vi "test_Antenna Pol Test.vi"(8 "error in (no error)":errorcluster, 11 "TestCase in":refnum<class "CO3000 Test Case.lvclass">) -> (0 "error out":errorcluster, 3 "TestCase out":refnum<class "CO3000 Test Case.lvclass">)   [LabVIEW 2020, in "CO3000 Test Case.lvclass"]
uses:
  CO3000 Test Case.lvclass
  CO3000 Test Case.lvclass/CO3000 Test Case.ctl
  CO3000.lvclass/CO3000.ctl
  CO3000.lvclass
  <vilib>/addons/_JKI Toolkits/VI Tester/TestCase.llb/TestCase.lvclass
  C:/Program Files (x86)/National Instruments/LabVIEW 2020/vi.lib/addons/_JKI Toolkits/VI Tester/TestCase.llb/TestCase.lvclass
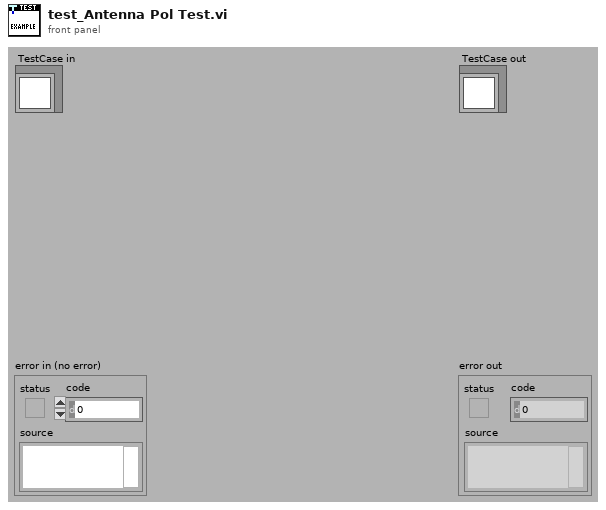
[diagram p1: front panel]
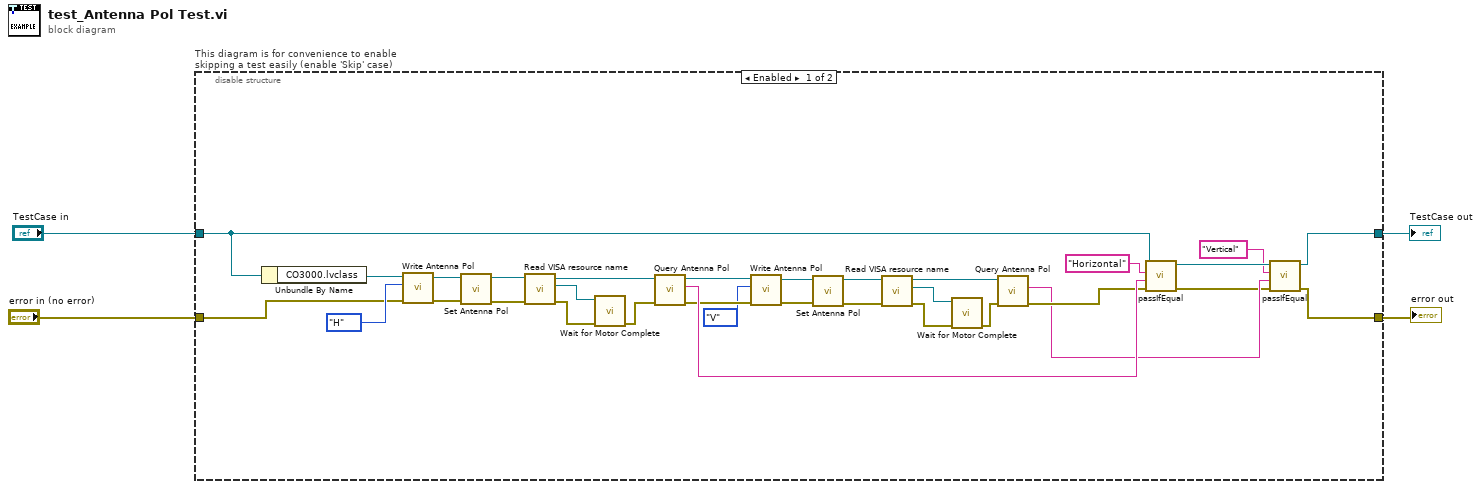
[diagram p0: block diagram]
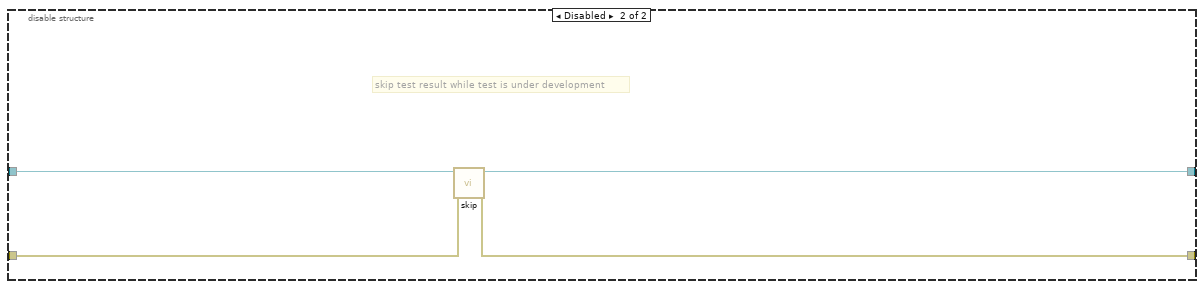
[diagram p2: hidden frame]
diagram:
  n1 = disable-structure "This diagram is for convenience to enable skipping a test easily (enable 'Skip' case)" shown="Enabled" {
    disable-tunnel: "TestCase in" -> [w36 w40]
    disable-tunnel: [w19 w38] -> w1
    disable-tunnel: [w15 w39] -> w3
    disable-tunnel: "error in (no error)" -> [w14 w37]
    frame Enabled {
      n2 = Unbundle By Name(w36) -> ("CO3000.lvclass"=w35:refnum<class "CO3000.lvclass">)
      n3 = call "Write Antenna Pol.vi"("error in (no error)"=w14, "Antenna Pol"=enum16{"H", "V"}."H", "CO3000 in"=w35) -> ("error out"=w32:errorcluster, "CO3000 out"=w33:refnum<class "CO3000.lvclass">)  [unwired: 7 in]
      n4 = call-dynamic "Set Antenna Pol.vi"("error in (no error)"=w32, "CO3000 in"=w33) -> ("error out"=w26:errorcluster, "CO3000 out"=w31:refnum<class "CO3000.lvclass">)  [unwired: 8 in]
      n5 = call "Read VISA resource name.vi"("error in (no error)"=w26, "CO3000 in"=w31) -> ("error out"=w27:errorcluster, "VISA resource name"=w30:refnum<visa-resource-name>, "CO3000 out"=w29:refnum<class "CO3000.lvclass">)  [unwired: 7 in]
      n6 = call "Wait for Motor Complete.vi"("error in (no error)"=w27, "VISA Refnum in"=w30) -> ("error out"=w28:errorcluster)  [unwired: 9 in]
      n7 = call-dynamic "Query Antenna Pol.vi"("error in (no error)"=w28, "CO3000 in"=w29) -> ("error out"=w22:errorcluster, "Antenna Pol"=w25:string, "CO3000 out"=w23:refnum<class "CO3000.lvclass">)  [unwired: 7 in]
      n8 = call "Write Antenna Pol.vi"("error in (no error)"=w22, "Antenna Pol"=enum16{"H", "V"}."V", "CO3000 in"=w23) -> ("error out"=w11:errorcluster, "CO3000 out"=w12:refnum<class "CO3000.lvclass">)  [unwired: 7 in]
      n9 = call-dynamic "Set Antenna Pol.vi"("error in (no error)"=w11, "CO3000 in"=w12) -> ("error out"=w7:errorcluster, "CO3000 out"=w8:refnum<class "CO3000.lvclass">)  [unwired: 8 in]
      n10 = call "Read VISA resource name.vi"("error in (no error)"=w7, "CO3000 in"=w8) -> ("error out"=w10:errorcluster, "VISA resource name"=w9:refnum<visa-resource-name>, "CO3000 out"=w5:refnum<class "CO3000.lvclass">)  [unwired: 7 in]
      n11 = call "Wait for Motor Complete.vi"("error in (no error)"=w10, "VISA Refnum in"=w9) -> ("error out"=w6:errorcluster)  [unwired: 9 in]
      n12 = call-dynamic "Query Antenna Pol.vi"("error in (no error)"=w6, "CO3000 in"=w5) -> ("error out"=w21:errorcluster, "Antenna Pol"=w17:string)  [unwired: 7 in, 1 out]
      n13 = call-dynamic "passIfEqual.vi"("error in (no error)"=w21, "y"=w25, "x"="Horizontal", "TestCase in"=w36) -> ("error out"=w16:errorcluster, "TestCase out"=w20:refnum<class "CO3000 Test Case.lvclass">)  [unwired: 6 in]
      n14 = call-dynamic "passIfEqual.vi"("error in (no error)"=w16, "y"=w17, "x"="Vertical", "TestCase in"=w20) -> ("error out"=w15:errorcluster, "TestCase out"=w19:refnum<class "CO3000 Test Case.lvclass">)  [unwired: 6 in]
    }
    frame Disabled {
      # "skip test result while test is under development"
      n15 = call <vilib>:"skip.vi"("error in (no error)"=w37, "TestCase in"=w40) -> ("error out"=w39:errorcluster, "TestCase out"=w38:refnum<class "CO3000 Test Case.lvclass">)  [unwired: 8 in]
    }
  }
  "error out" <- w3
  "TestCase out" <- w1
